vi "Measure Inband.vi"(8 "error in (no error)":errorcluster caption="에러 입력(에러 없음)", 11 "Instrument Manager 입력":refnum<class "Instrument Manager.lvclass">) -> (0 "error out":errorcluster caption="에러 출력", 2 "Y-axis":dbl, 3 "Instrument Manager 출력":refnum<class "Instrument Manager.lvclass">)   [LabVIEW 2023, in "Instrument Manager.lvclass"]
uses:
  Instrument Manager.lvclass
  Instrument Manager.lvclass/Instrument Manager.ctl
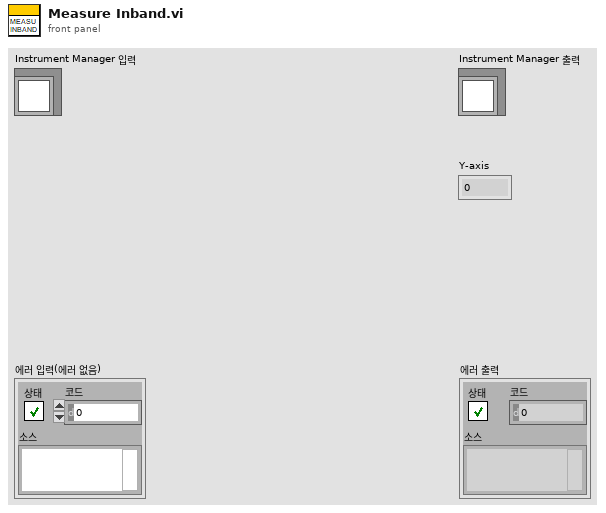
[diagram p1: front panel]
types:
  T1 = typedef "Spectrum Analyzer.lvlib/TYPE Marker Value.ctl" = cluster{"X-axis":dbl, "Y-axis":dbl}
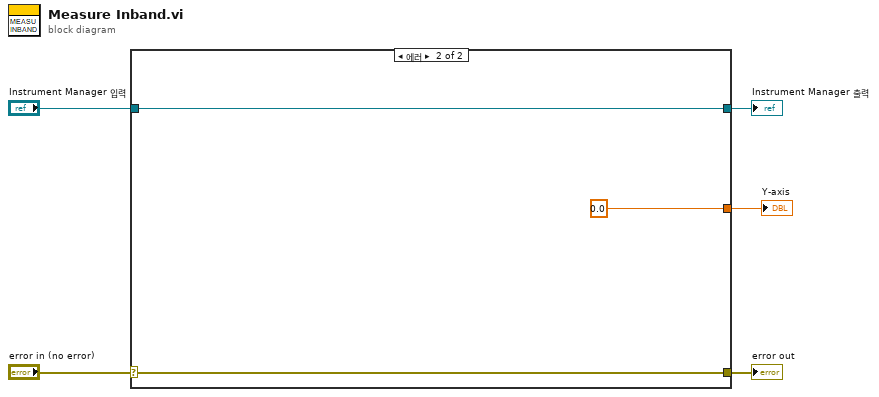
[diagram p0: block diagram]
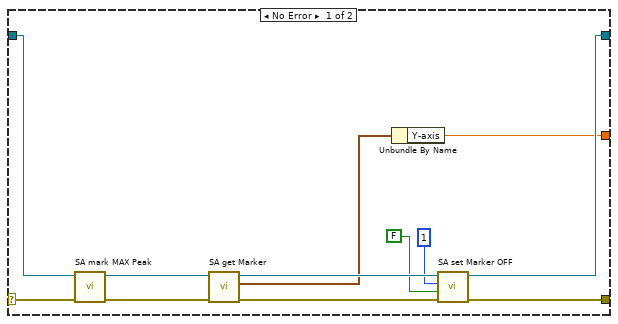
[diagram p2: hidden frame]
diagram:
  n1 = case shown="에러" "error in (no error)" {
    selector: "error in (no error)" -> [w10 w20]
    tunnel: [w9 w20] -> w4
    tunnel: [w8 w19] -> w2
    tunnel: "Instrument Manager 입력" -> [w13 w19]
    tunnel: [w6 0.0 ("Y-axis")] -> w1
    frame No Error {
      n2 = call "SA mark MAX Peak.vi"("error in (no error)"=w10, "Instrument Manager 입력"=w13) -> ("error out"=w17:errorcluster, "Instrument Manager 출력"=w16:refnum<class "Instrument Manager.lvclass">)  [unwired: 8 in]
      n3 = call "SA get Marker.vi"("error in (no error)"=w17, "Instrument Manager 입력"=w16) -> ("error out"=w15:errorcluster, "Marker Value"=w7:T1, "Instrument Manager 출력"=w14:refnum<class "Instrument Manager.lvclass">)  [unwired: 7 in]
      n4 = Unbundle By Name(w7) -> ("Y-axis"=w6:dbl)
      n5 = call "SA set Marker OFF.vi"("error in (no error)"=w15, "On?"=FALSE, "Marker Index"=1, "Instrument Manager 입력"=w14) -> ("error out"=w9:errorcluster, "Instrument Manager 출력"=w8:refnum<class "Instrument Manager.lvclass">)  [unwired: 6 in]
    }
    frame Error {
    }
  }
  "error out" <- w4
  "Instrument Manager 출력" <- w2
  "Y-axis" <- w1
